vi "ubidots envia_recibe.vi"() -> ()   [LabVIEW 2019]
uses:
  <vilib>/Instr/_visa.llb/VISA Configure Serial Port (Instr).vi
panel:
  in  "VISA resource name":refnum<visa-resource-name>
  out "data out 3":string
  out "pwm":dbl(knob) scale=0.0..255.0
  out "concatenated string 3":string
  out "data out 2":string
  out "suiche":bool
  out "concatenated string":string
  in  "LED":bool
  in  "Temperatura":dbl(slide) scale=0.0..100.0
  in  "stop":bool
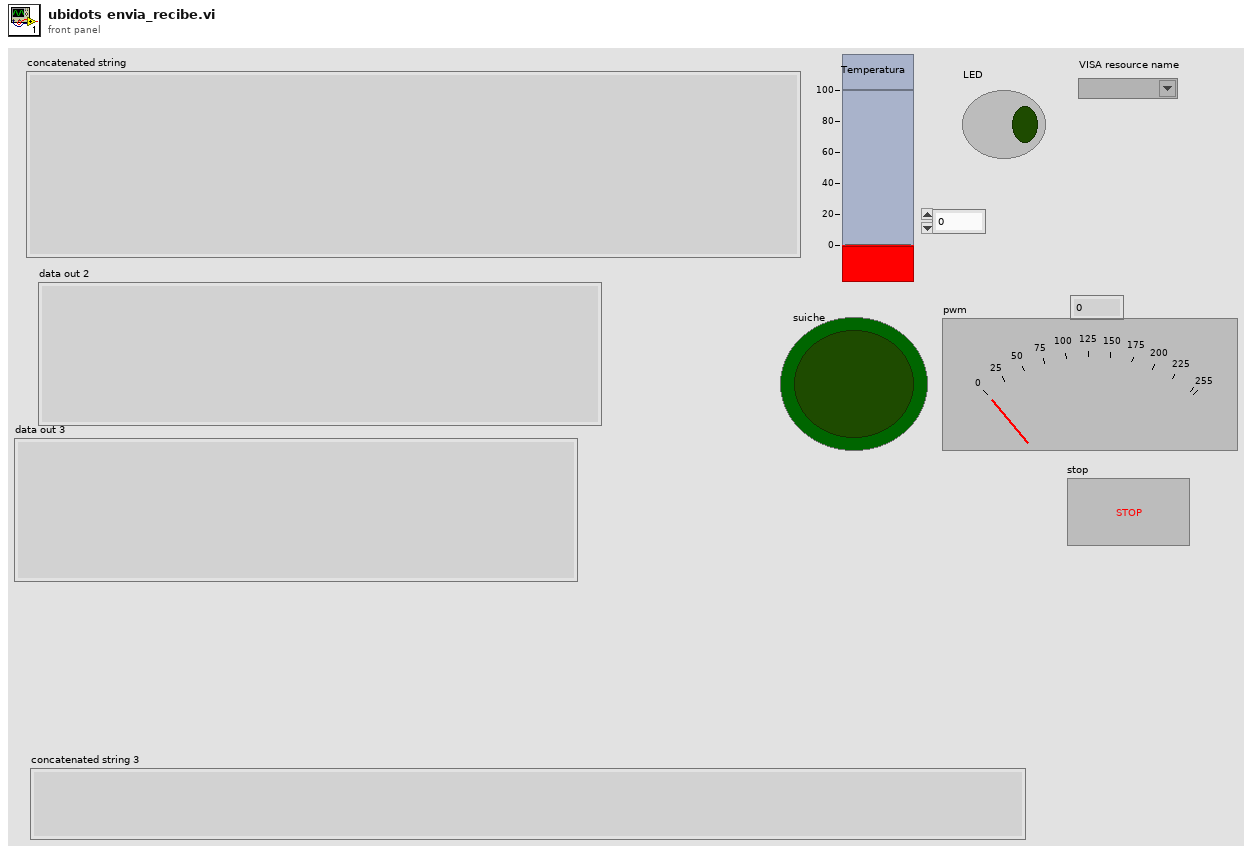
[diagram p1: front panel]
types:
  T1 = enum16{"Standard", "Buffered", "CRLF", "Immediate"}
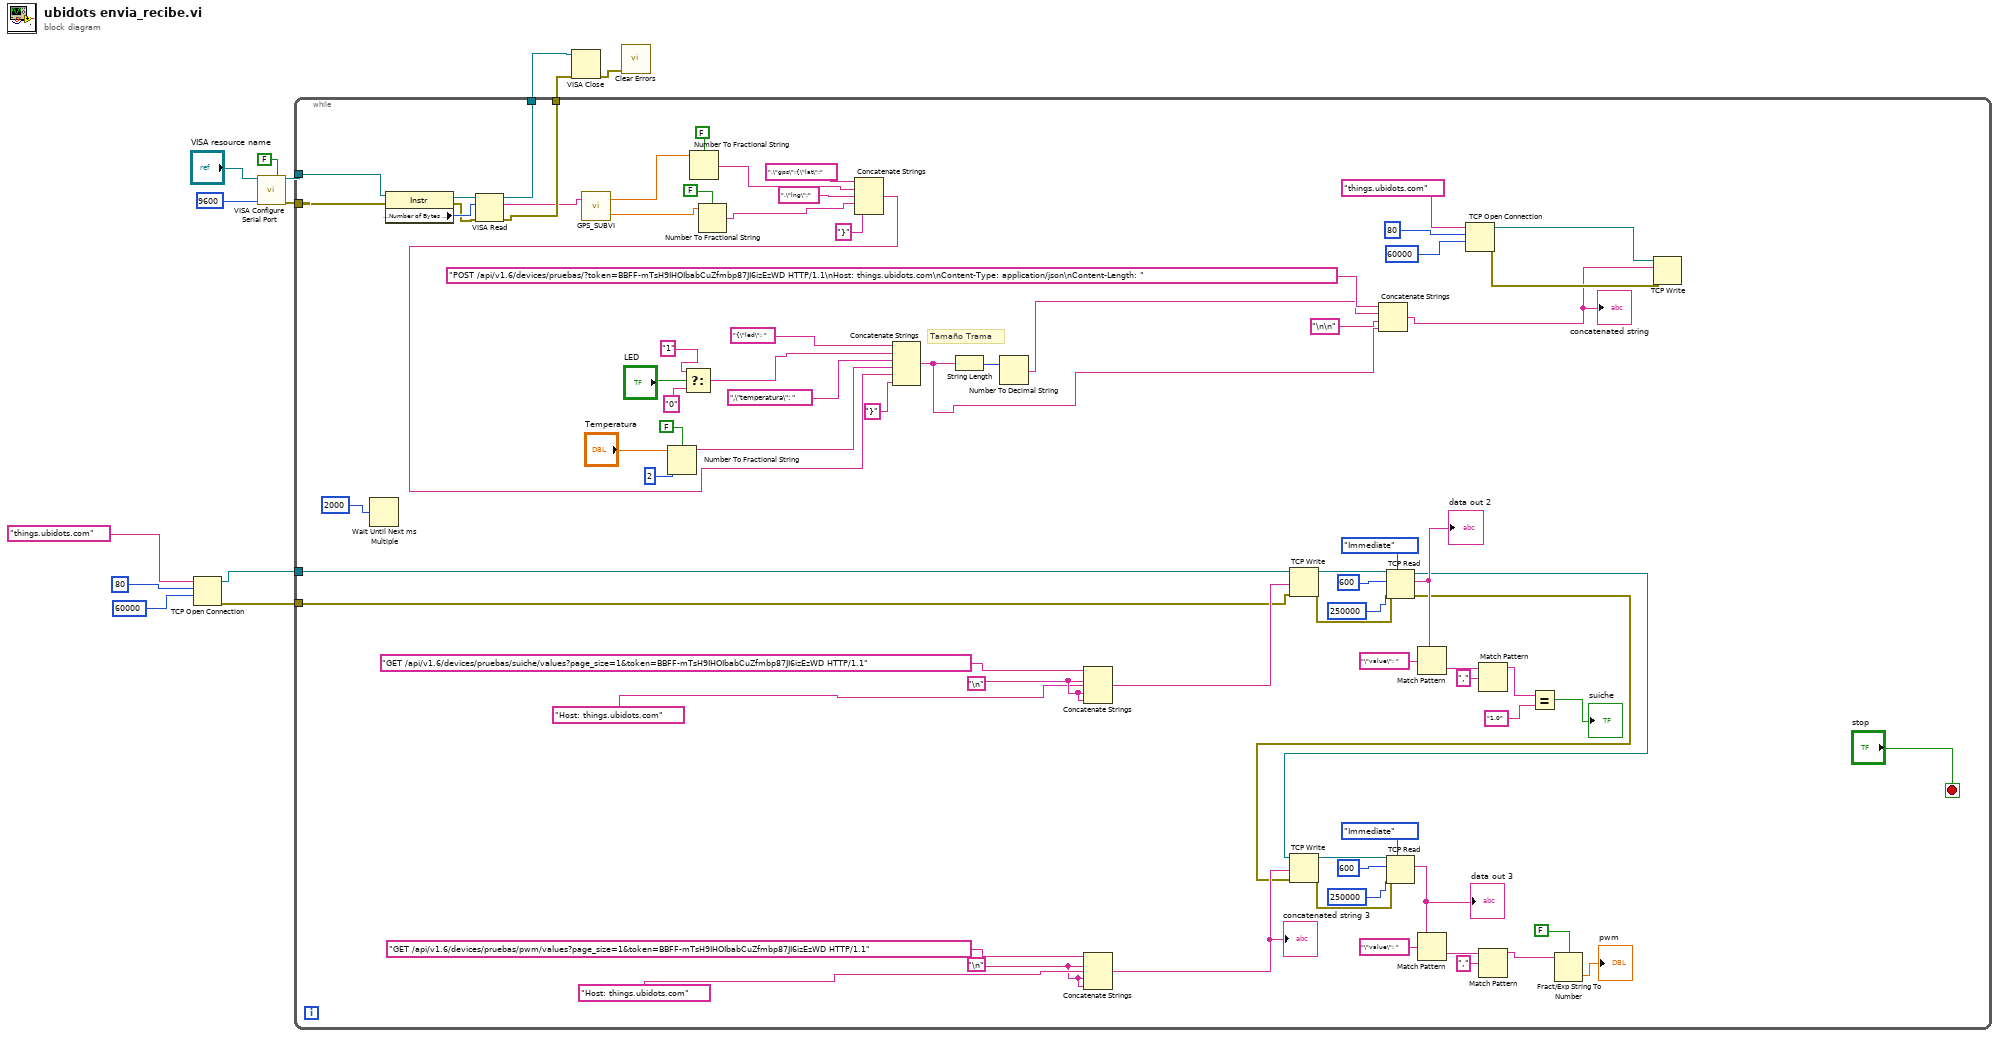
[diagram p0: block diagram]
diagram:
  n1 = TCP Open Connection(address="things.ubidots.com", remote port or service name=u16 80, timeout ms (60000)=60000) -> (connection ID=w10:refnum<k5>, error out=w9:errorcluster)  [unwired: 2 in]
  n2 = call-poly "VISA Configure Serial Port"("VISA resource name"="VISA resource name", "Enable Termination\nChar (T)"=FALSE ("Enable Termination\nChar (T)"), "baud rate (9600)"=u32 9600) -> ("VISA resource name out"=w8:refnum<visa-resource-name>, "error out"=w7:errorcluster)  [unwired: 11 in]
  n3 = while {
    tunnel: w10 -> [w54]
    tunnel: w9 -> [w53]
    tunnel: w8 -> [w32]
    tunnel: w7 -> [w31]
    tunnel: [w27] -> w3
    tunnel: [w26] -> w2
    stop <- "stop" stop-if-true
    w42 = "\n"
    w63 = "\n"
    # "Tamaño Trama"
    n4 = Wait Until Next ms Multiple(millisecond multiple=u32 2000 ("milliseconds to wait")) -> ()  [unwired: 1 out]
    n5 = property class="Instr"(reference=w32, error in=w31) -> (reference out=w30:refnum<visa-resource-name>, error out=w28:errorcluster, "Serial Settings:Number of Bytes at Serial Port"=w29:u32)
    n6 = VISA Read(VISA resource name=w30, byte count=w29, error in (no error)=w28) -> (VISA resource name out=w27:refnum<visa-resource-name>, read buffer=w25:string, error out=w26:errorcluster)  [unwired: 1 out]
    n7 = call "GPS_SUBVI.vi"("String"=w25) -> ("LONGITUD"=w23:dbl, "LATITUD"=w24:dbl)  [unwired: 1 in]
    n8 = Number To Fractional String(use system decimal point (T)=FALSE, number="Temperatura", precision (6)=i16 2) -> (F-format string=w76:string)  [unwired: 1 in]
    n9 = Select(t="1" ("string"), s="LED", f="0" ("string")) -> (s? t:f=w80:string)
    n10 = Number To Fractional String(use system decimal point (T)=FALSE, number=w24) -> (F-format string=w18:string)  [unwired: 2 in]
    n11 = Number To Fractional String(use system decimal point (T)=FALSE, number=w23) -> (F-format string=w16:string)  [unwired: 2 in]
    n12 = Concatenate Strings(",\"gps\":{\"lat\":" ("string"), w18, ",\"lng\":" ("string"), w16, "}" ("string")) -> (w14:string)
    n13 = Concatenate Strings("{\"led\": " ("string"), w80, ",\"temperatura\": " ("string"), w76, w14, "}" ("string")) -> (w72:string)
    n14 = String Length(string=w72) -> (length=w75:i32)
    n15 = Number To Decimal String(number=w75) -> (decimal integer string=w74:string)  [unwired: 1 in]
    n16 = Concatenate Strings("GET /api/v1.6/devices/pruebas/suiche/values?page_size=1&token=BBFF-mTsH9IHOIbabCuZfmbp87JI6izEzWD HTTP/1.1" ("data in"), w63, "Host: things.ubidots.com" ("string"), w63, w63) -> (w61:string)
    n17 = Concatenate Strings("GET /api/v1.6/devices/pruebas/pwm/values?page_size=1&token=BBFF-mTsH9IHOIbabCuZfmbp87JI6izEzWD HTTP/1.1" ("data in"), w42, "Host: things.ubidots.com" ("string"), w42, w42) -> (w44:string)
    "concatenated string 3" <- w44
    n18 = TCP Write(connection ID=w54, data in=w61, error in (no error)=w53) -> (connection ID out=w58:refnum<k5>, error out=w57:errorcluster)  [unwired: 1 in, 1 out]
    n19 = Concatenate Strings("POST /api/v1.6/devices/pruebas/?token=BBFF-mTsH9IHOIbabCuZfmbp87JI6izEzWD HTTP/1.1\nHost: things.ubidots.com\nContent-Type: application/json\nContent-Length: " ("string"), w74, "\n\n" ("string"), w72) -> (w71:string)
    "concatenated string" <- w71
    n20 = TCP Read(connection ID=w58, bytes to read=600, error in (no error)=w57, 7:T1."Immediate" ("mode (standard)"), 9:250000 ("timeout ms (25000)")) -> (connection ID out=w38:refnum<k5>, data out=w64:string, error out=w37:errorcluster)
    "data out 2" <- w64
    n21 = TCP Write(connection ID=w38, data in=w44, error in (no error)=w37) -> (connection ID out=w47:refnum<k5>, error out=w48:errorcluster)  [unwired: 1 in, 1 out]
    n22 = TCP Read(connection ID=w47, bytes to read=600, error in (no error)=w48, 7:T1."Immediate" ("mode (standard)"), 9:250000 ("timeout ms (25000)")) -> (data out=w34:string)  [unwired: 2 out]
    "data out 3" <- w34
    n23 = Match Pattern(string=w64, regular expression="\"value\": ") -> (after substring=w66:string)  [unwired: 1 in, 3 out]
    n24 = Match Pattern(string=w34, regular expression="\"value\": ") -> (after substring=w40:string)  [unwired: 1 in, 3 out]
    n25 = TCP Open Connection(address="things.ubidots.com", remote port or service name=u16 80, timeout ms (60000)=60000) -> (connection ID=w88:refnum<k5>, error out=w89:errorcluster)  [unwired: 2 in]
    n26 = Match Pattern(string=w66, regular expression=",") -> (before substring=w68:string)  [unwired: 1 in, 3 out]
    n27 = Match Pattern(string=w40, regular expression=",") -> (before substring=w35:string)  [unwired: 1 in, 3 out]
    n28 = Equal?(x=w68, y="1.0") -> (x = y?=→"suiche":bool)
    n29 = Fract/Exp String To Number(use system decimal point (T)=FALSE, string=w35) -> (number=→"pwm":dbl)  [unwired: 2 in, 1 out]
    n30 = TCP Write(connection ID=w88, data in=w71, error in (no error)=w89) -> ()  [unwired: 1 in, 3 out]
  }
  n31 = VISA Close(VISA resource name=w3, error in (no error)=w2) -> (error out=w1:errorcluster)
  n32 = call <vilib>:"Clear Errors.vi"("error in (no error)"=w1) -> ()  [unwired: 5 in, 2 out]
